vi "Example 02b - Lua Scripts with Arguments.vi"() -> ()   [LabVIEW 2020]
uses:
  Lua for LabVIEW/Lua/Lua.lvclass
panel:
  out "-number":dbl
  out "-integer":i64
  out "!boolean":bool
  out "upper(string)":string
  in  "an_integer":i64=58812
  in  "a boolean":bool=TRUE
  in  "a string":string="my name is ..."
  in  "a double":dbl=2.2
  out "error out":errorcluster
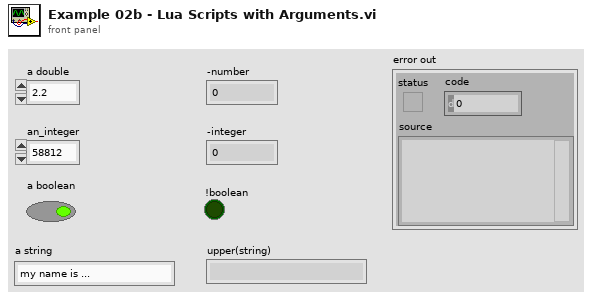
[diagram p1: front panel]
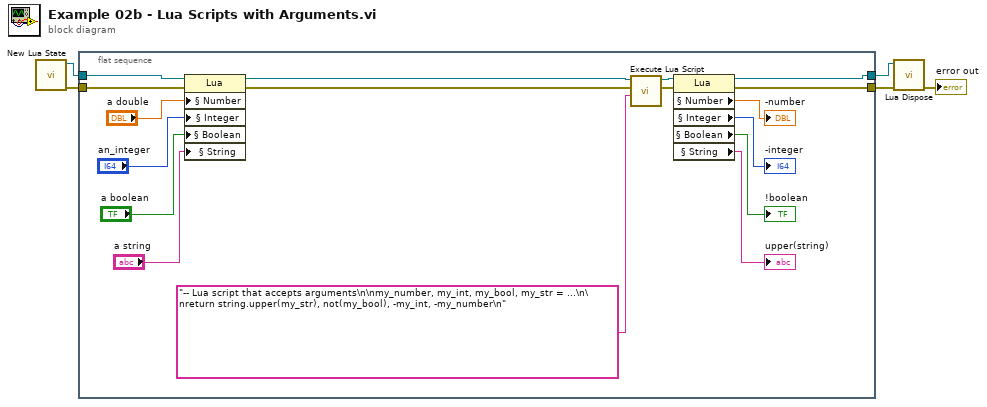
[diagram p0: block diagram]
diagram:
  n1 = call "New Lua State.vi"() -> ("error out"=w4:errorcluster, "Lua out"=w5:refnum<class "Lua.lvclass">)  [unwired: 10 in]
  n2 = flat-sequence {
    tunnel: w5 -> [w18]
    tunnel: w4 -> [w17]
    tunnel: [w21] -> w2
    tunnel: [w20] -> w1
    frame #0 {
      n3 = property class="Lua"(reference=w18, error in=w17, "§ Number"="a double", "§ Integer"="an_integer", "§ Boolean"="a boolean", "§ String"="a string") -> (reference out=w19:refnum<class "Lua.lvclass">, error out=w8:errorcluster)
      n4 = call-dynamic "Execute Lua Script.vi"("lua script"="-- Lua script that accepts arguments\n\nmy_number, my_int, my_bool, my_str = ...\n\nreturn string.upper(my_str), not(my_bool), -my_int, -my_number\n", "error in (no error)"=w8, "Lua in"=w19) -> ("error out"=w6:errorcluster, "Lua out"=w22:refnum<class "Lua.lvclass">)  [unwired: 7 in]
      n5 = property class="Lua"(reference=w22, error in=w6) -> (reference out=w20:refnum<class "Lua.lvclass">, error out=w21:errorcluster, "§ Number"=→"-number":dbl, "§ Integer"=→"-integer":i64, "§ Boolean"=→"!boolean":bool, "§ String"=→"upper(string)":string)
    }
  }
  n6 = call-dynamic "Lua Dispose.vi"("error in (no error)"=w2, "Lua in"=w1) -> ("error out"=→"error out":errorcluster)  [unwired: 9 in]
